vi "Example Edge Detect.vi"() -> ()   [LabVIEW 2025]
uses:
  wiringPi.lvlib
  Type Defs/GPIO Pins.ctl
  Type Defs/Pull up-down.ctl
  GPIO/Internal/waitForInterrupt.Both.vi
  GPIO/Internal/pinMode.Input.vi
  Type Defs/Edge Mode.ctl
panel:
  out "Detected Edge":T1=enum."Edge Falling"
  out "stoping":bool
  in  "stop":bool
  out "Detected":bool
  in  "Value Write":bool
  out "Value Read":bool
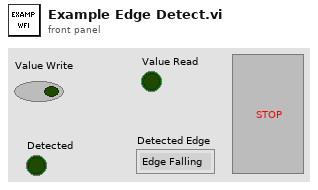
[diagram p1: front panel]
types:
  T1 = typedef "wiringPi.lvlib/Edge Mode.ctl" = enum32{"None", "Edge Falling", "Edge Rising", "Both"}
  T2 = typedef "wiringPi.lvlib/GPIO Pins.ctl" = enum32{"GPIO0_I2C0_SDA_Pin27", "GPIO1_I2C0_SDA1_Pin28", "GPIO2_I2C1_SDA_Pin3", "GPIO3_I2C1_SCL_Pin5", "GPIO4_GPCLK0_Pin7", "GPIO5_GPCLK1_Pin29", "GPIO6_GPCLK2_Pin31", "GPIO7_SPI_CE1_N_Pin26", "GPIO8_SPI_CE0_N_Pin24", "GPIO9_SPI0_MISO_Pin21", "GPIO10_SPI0_MOSI_Pin19", "GPIO11_SPI0_CLK_Pin23", "GPIO12_PWM0_Pin32", "GPIO13_PWM1_Pin33", "GPIO14_TXD0_Pin8", "GPIO15_RXD0_Pin10", "GPIO16_Pin36", "GPIO17_Pin11", "GPIO18_PWM0_Pin12", "GPIO19_PWM1_Pin35", "GPIO20_GPCLK0_Pin38", "GPIO21_GPCLK1_Pin40", "GPIO22_Pin15", "GPIO23_Pin16", "GPIO24_Pin18", "GPIO25_Pin22", "GPIO26_Pin37", "GPIO27_Pin13"}
  T3 = typedef "wiringPi.lvlib/Pull up-down.ctl" = enum16{"Off", "Down", "Up"}
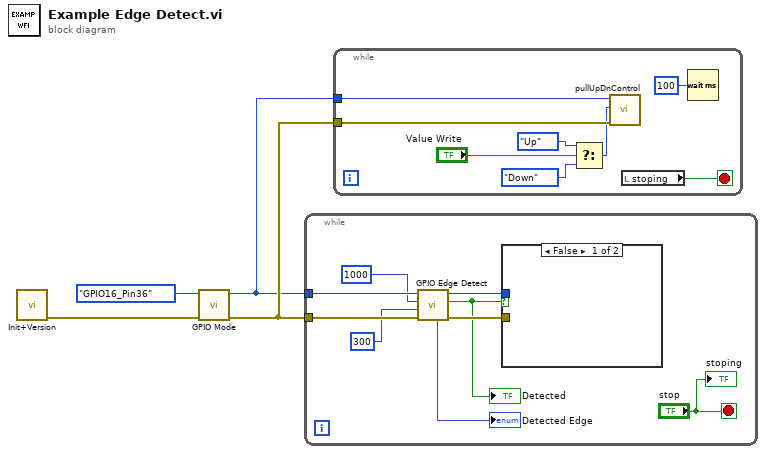
[diagram p0: block diagram]
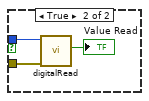
[diagram p2: hidden frame]
diagram:
  n1 = call "Init+Version.vi"() -> ("error out"=w3:errorcluster)  [unwired: 8 in, 3 out]
  n2 = call-poly "GPIO Mode.vi"("error in (no error)"=w3, "RPi Pin"=GPIO_Pins."GPIO16_Pin36") -> ("error out"=w2:errorcluster, "RPi Pin out"=w1:T2)  [unwired: 8 in]
  n3 = while {
    tunnel: w2 -> [w12]
    tunnel: w1 -> [w13]
    stop <- "stop" stop-if-true
    n4 = call-poly "GPIO Edge Detect.vi"("error in (no error)"=w12, "Debounce (us)"=u32 300 ("debounce_period_us"), "Timeout (ms)"=1000 ("ms"), "RPi Pin"=w13) -> ("error out"=w11:errorcluster, "Detected"=w7:bool, "RPi Pin out"=w10:T2, "Detected Edge"=→"Detected Edge":T1)  [unwired: 3 in, 1 out]
    "Detected" <- w7
    n5 = case shown="False" w7 {
      tunnel: w11 -> [_ w15]
      tunnel: w10 -> [_ w14]
      frame False {
      }
      frame True {
        n6 = call "digitalRead.vi"("error in (no error)"=w15, "RPi Pin"=w14) -> ("Value"=→"Value Read":bool)  [unwired: 7 in, 2 out]
      }
    }
    "stoping" <- "stop"
  }
  n7 = while {
    tunnel: w2 -> [w24]
    tunnel: w1 -> [w23]
    stop <- w17 stop-if-true
    n8 = Select(t=Pull_up-down."Up" ("Up-Down-Off"), s="Value Write", f=Pull_up-down."Down") -> (s? t:f=w18:T3)
    n9 = call "pullUpDnControl.vi"("error in (no error)"=w24, "Up-Down-Off"=w18, "RPi Pin"=w23) -> ()  [unwired: 7 in, 2 out]
    n10 = local read "stoping"() -> (w17:bool)
    n11 = Wait (ms)(milliseconds to wait=u32 100) -> ()  [unwired: 1 out]
  }
